vi "crop_coin_planar.vi"(4 "height":sgl, 6 "width":sgl, 7 "pad Color":u32(colorbox)=7500402, 8 "error in (no error)":errorcluster, 9 "center_y":sgl, 10 "center_x":sgl, 11 "image in":T1) -> (0 "error out":errorcluster, 1 "is_fully_visible":i32, 3 "image out":T1)   [LabVIEW 2018, in "Image Processing Library.lvlib"]
uses:
  Image Processing Library.lvlib
  <vilib>/picture/picture.llb/imagedata.ctl
panel:
  out "crop_h":i32
  out "crop_w":i32
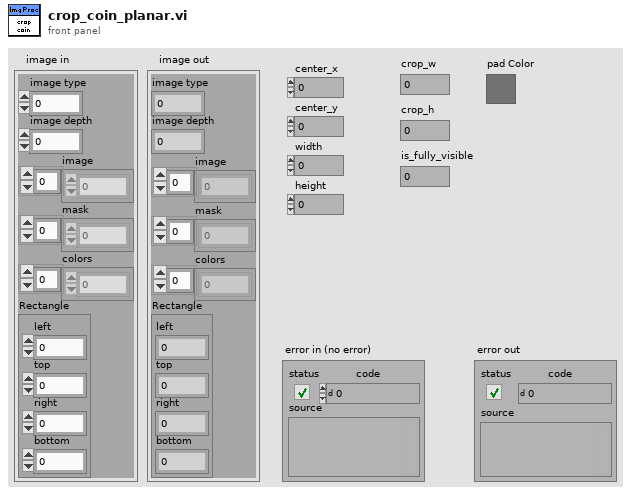
[diagram p1: front panel]
types:
  T1 = typedef "imagedata.ctl" = cluster{"image type":i32, "image depth":i32, "image":u8[], "mask":u8[], "colors":u32[], "Rectangle":cluster{"left":i16, "top":i16, "right":i16, "bottom":i16}}
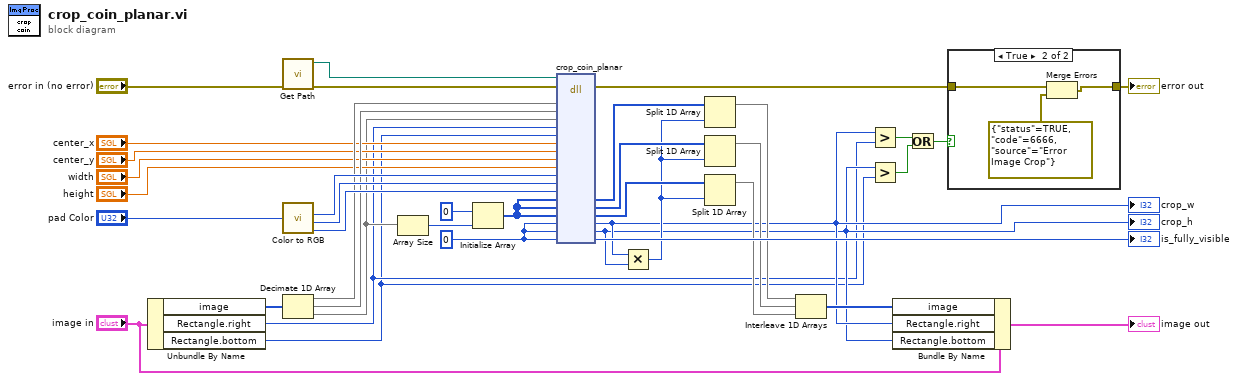
[diagram p0: block diagram]
diagram:
  w19 = 0 ("out_left")
  n1 = Unbundle By Name("image in") -> ("image"=w29:u8[], "Rectangle.right"=w7:i16, "Rectangle.bottom"=w6:i16)
  n2 = call "Get Path.vi"("error in (no error)"="error in (no error)") -> ("error out"=w38:errorcluster, "Library Path"=w37:path)  [unwired: 9 in]
  n3 = call <vilib>:"Color to RGB.vi"("Color"="pad Color") -> ("R"=w35:u8, "G"=w34:u8, "B"=w33:u8)  [unwired: 1 out]
  n4 = Decimate 1D Array(w29) -> (w28:u8[], w27:u8[], w10:u8[])
  n5 = Array Size(array=w10) -> (size(s)=w11:i32)
  n6 = Initialize Array(u8 0 ("element"), w11) -> (w30:u8[])
  n7 = dll-call lib="D:/Astra/LabVIEWData/ONNX/Coin Detector/Project_2018/image_processing/windows_x64/image_processing.dll" fn="crop_coin_planar"(path in=w37, error in=w38, "in_r"=w28, "in_g"=w27, "in_b"=w10, "orig_w"=w7, "orig_h"=w6, "center_x"="center_x", "center_y"="center_y", "width"="width", "height"="height", "pad_r"=w35, "pad_g"=w34, "pad_b"=w33, "out_r"=w30, "out_g"=w30, "out_b"=w30, "crop_w"=w19, "crop_h"=w19, "is_fully_visible"=w19) -> (error out=w2:errorcluster, "out_r"=w18:u8[], "out_g"=w17:u8[], "out_b"=w16:u8[], "crop_w"=w9:i32, "crop_h"=w8:i32, "is_fully_visible"=→"is_fully_visible":i32)  [unwired: 14 in, 1 out]
  "crop_w" <- w9
  "crop_h" <- w8
  n8 = Multiply(x=w9, y=w8) -> (x*y=w15:i32)
  n9 = Split 1D Array(array=w18, index=w15) -> (first subarray=w13:u8[])  [unwired: 1 out]
  n10 = Split 1D Array(array=w17, index=w15) -> (first subarray=w14:u8[])  [unwired: 1 out]
  n11 = Split 1D Array(array=w16, index=w15) -> (first subarray=w12:u8[])  [unwired: 1 out]
  n12 = Interleave 1D Arrays(w13, w14, w12) -> (w26:u8[])
  n13 = Greater?(x=w9, y=w7) -> (0:w5:bool)
  n14 = Greater?(x=w8, y=w6) -> (0:w4:bool)
  n15 = Bundle By Name(cluster="image in", "image"=w26, "Rectangle.right"=w9, "Rectangle.bottom"=w8) -> (→"image out":T1)
  n16 = Or(x=w5, y=w4) -> (x .or. y?=w3:bool)
  n17 = case shown="True" w3 {
    tunnel: w2 -> [w40 w43]
    tunnel: [w40 w42] -> w1
    frame False {
    }
    frame True {
      n18 = Merge Errors(w43, errorcluster {"status"=TRUE, "code"=6666, "source"="Error Image Crop"} ("error in")) -> (w42:errorcluster)
    }
  }
  "error out" <- w1
